vi "AR Drone - Simple Video + Simple nav.vi"() -> ()   [LabVIEW 2014]
doc: "Very simple example showing how to use the base VIs to control the AR Drone and receive and display video data."
uses:
  AR Drone - Simple Video + Simple nav Folder/Control cluster.ctl
  <vilib>/LVH/AR Drone Toolkit/Decode NavData/Typedefs/NavData Demo.ctl
  Global.vi
  <vilib>/LVH/AR Drone Toolkit/AR Drone.lvlib
panel:
  in  "Tab Control 2":enum32{"Setup", "Debug&Test Info", "NavData"}(tab)
  in  "Setup Parameters":T1={"Drone IP address"="192.168.1.1", "Home IP address"="192.168.1.2", "Flight Mode"=enum."INDOOR MODE", "Mounted Hull"=enum."INDOOR HULL", "Video Camera"=1, "Max Altitude (m)"=3.0, "Max Pitch and Roll Angle (deg)"=8.0, "Max Vertical Speed (m/s)"=0.7, "Max Yaw Speed (deg/s)"=100.0} {"Video Camera" items=["Bottom Camera"=1, "Front Camera"=0, "Front in Bottom"=3, "Bottom in Front"=2]}
  in  "device ID":i32=3
  in  "Video Acquisition VI path":path=path "Video Processing.vi"
  in  "Adjustments":cluster{"Sensitivity":dbl, "Null Zone":dbl}={"Sensitivity"=1.0, "Null Zone"=1.0} {"Null Zone" scale=0.0..5.0; "Sensitivity" scale=0.0..5.0}
  out "ctr+nav 2":i32=2242
  in  "milliseconds to wait":u32=10
  out "Refesh Rate (ms)":u32=5
  out "Refesh Rate Video Loop (ms) 2":u32
  in  "video refresh (ms)":u32=40
  out "ctr+nav":errorcluster
  out "NavData Out 2":T2={"control state"=enum."TRANS_LANDING", "battery percentage"=55, "pitch (deg)"=-0.02, "roll (deg)"=0.087, "yaw (deg)"=91.646, "altitude (cm)"=0, "vx (cm/s)?"=0.0, "vy (cm/s)?"=0.0, "vz (cm/s)?"=0.0, "detection cam type"=3}
  out "Battery Remaining 2":dbl(slide)=55.0 scale=0.0..100.0
  out "Hover":bool
  out "Control Cluster":T3={"Roll"=0.0, "Pitch"=-0.10223389, "Vertical Speed"=0.0, "Yaw Speed"=0.0} {"Yaw Speed" scale=-1.0..1.0; "Vertical Speed" scale=-1.0..1.0; "Pitch" scale=-1.0..1.0; "Roll" scale=-1.0..1.0}
  out "error":bool
  out "Take off/Land":bool
  in  "Tab Control":enum32{"Raw Image", "Grayscale", "Black&White"}(tab)
  out "Raw":picture
  out "Grayscale":T4(plugin-control)
  out "B&W":T4(plugin-control)
  in  "Manual":bool=TRUE
  in  "stop":bool
  in  "Emergency Landing":bool
  # "(1 is default)"
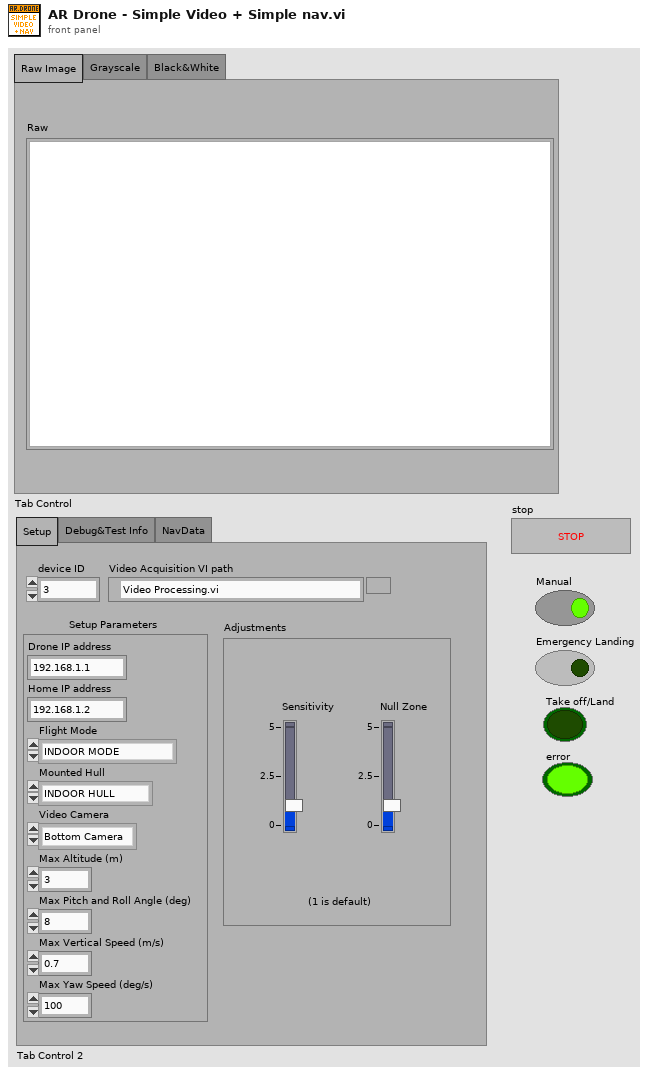
[diagram p1: front panel]
types:
  T1 = cluster{"Drone IP address":string, "Home IP address":string, "Flight Mode":enum8{"OUTDOOR MODE", "INDOOR MODE"}, "Mounted Hull":enum8{"OUTDOOR HULL", "INDOOR HULL"}, "Video Camera":u8, "Max Altitude (m)":sgl, "Max Pitch and Roll Angle (deg)":sgl, "Max Vertical Speed (m/s)":sgl, "Max Yaw Speed (deg/s)":sgl}
  T2 = typedef "AR Drone.lvlib/NavData Demo.ctl" = cluster{"control state":enum32{"DEFAULT", "INIT", "LANDING", "FLYING", "HOVERING", "TEST", "TRANS_TAKEOFF", "TRANS_GOTOFIX", "TRANS_LANDING"}, "battery percentage":u32, "pitch (deg)":sgl, "roll (deg)":sgl, "yaw (deg)":sgl, "altitude (cm)":u32, "vx (cm/s)?":sgl, "vy (cm/s)?":sgl, "vz (cm/s)?":sgl, "detection cam type":u32}
  T3 = typedef "Control cluster.ctl" = cluster{"Roll":sgl, "Pitch":sgl, "Vertical Speed":sgl, "Yaw Speed":sgl}
  T4 = typedef "IMAQ Image.ctl" = refnum<image>
  T5 = typedef "AR Drone.lvlib/AR Drone Resource.ctl" = cluster{"UDP Control Connection":refnum<k16>, "UDP NavData Connection":refnum<k16>, "UDP Video Connection (Drone 1.0)":refnum<k16>, "TCP Video Connection (Drone 2.0)":refnum<k5>, "TCP Control Port Connection":refnum<k5>, "Drone IP address":string, "Drone Command Port":u16, "Drone NavData Port":u16, "Drone Vid Stream Port":u16, "Drone TCP Control Port":u16, "Home IP address":string, "Home Command Port":u16, "Home NavData Port":u16, "Home Vid Stream Port":u16, "Drone Version":i32, "Drone Index":i32, "Command Sequence":i32}
  T6 = cluster{"Hover":bool, "Land/Take off":bool, "button 3":bool, "button 4":bool}
  T7 = cluster{"Roll":dbl, "Pitch":dbl, "Vertical Speed":dbl, "Yaw Speed":dbl}
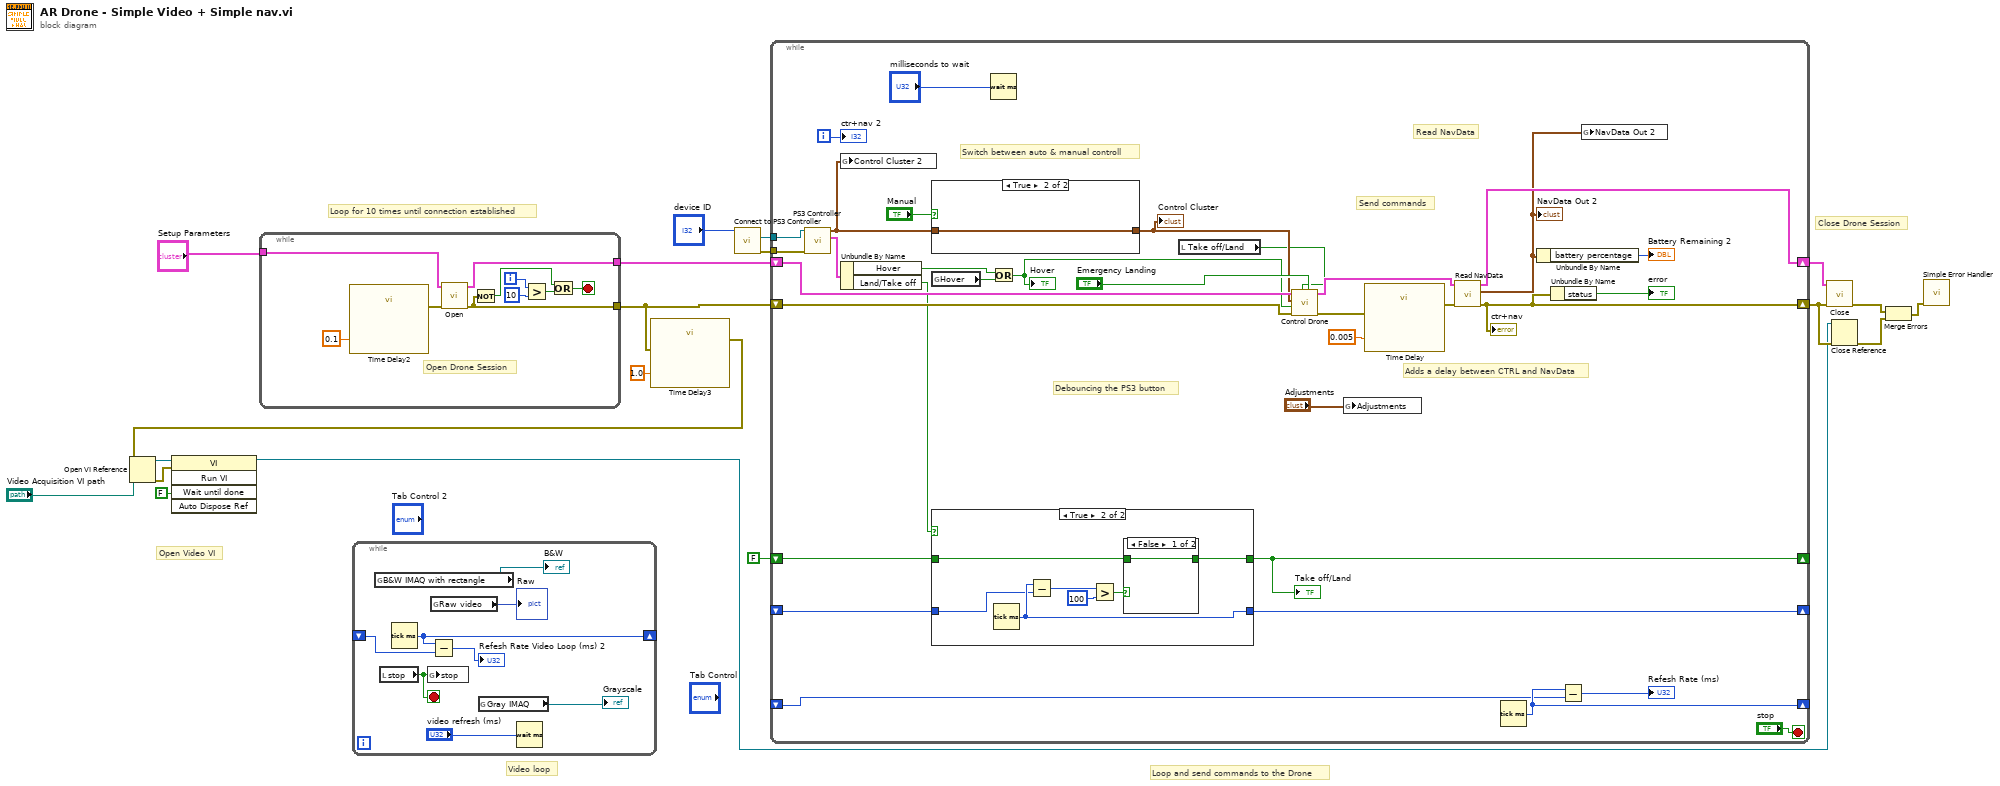
[diagram p0: block diagram]
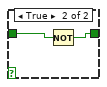
[diagram p3: hidden frame]
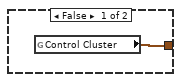
[diagram p4: hidden frame]
diagram:
  # "Open Video VI"
  # "Loop for 10 times until connection established"
  # "Video loop"
  # "Close Drone Session"
  # "Loop and send commands to the Drone"
  n1 = while {
    tunnel: [w21] -> w13
    tunnel: "Setup Parameters" -> [w29]
    tunnel: [w20] -> w5
    i -> [w25]
    stop <- w27 stop-if-true
    # "Open Drone Session"
    n2 = call "Time Delay2"("Delay Time (s)"=0.1) -> ("error out"=w22:errorcluster)  [unwired: 10 in]
    n3 = call <vilib>:"Open.vi"("error in (no error)"=w22, "Setup Parameters"=w29) -> ("error out"=w21:errorcluster, "AR Drone Resource"=w20:T5)  [unwired: 8 in]
    n4 = Not(x=w21) -> (.not. x?=w23:bool)
    n5 = Greater?(x=w25, y=10) -> (0:w26:bool)
    n6 = Or(x=w23, y=w26) -> (x .or. y?=w27:bool)
  }
  n7 = while {
    shift-right: [w35] -> _
    shift-left: _ -> [w34]
    stop <- w31 stop-if-true
    n8 = global read "Global.vi" "B&W IMAQ with rectangle"() -> (→"B&W":T4)
    n9 = local read "stop"() -> (w31:bool)
    n10 = Tick Count (ms)() -> (millisecond timer value=w35:u32)
    n11 = global write "Global.vi" "stop"(w31) -> ()
    n12 = global read "Global.vi" "Raw video"() -> (→"Raw":picture)
    n13 = Subtract(x=w35, y=w34) -> (x-y=→"Refesh Rate Video Loop (ms) 2":u32)
    n14 = global read "Global.vi" "Gray IMAQ"() -> (→"Grayscale":T4)
    n15 = Wait (ms)(milliseconds to wait="video refresh (ms)") -> ()  [unwired: 1 out]
  }
  n16 = call "Time Delay3"("error in (no error)"=w13, "Delay Time (s)"=1.0) -> ("error out"=w1:errorcluster)  [unwired: 9 in]
  n17 = Open VI Reference(vi path="Video Acquisition VI path", error in (no error)=w1) -> (vi reference=w9:refnum<vi>, error out=w7:errorcluster)  [unwired: 4 in]
  n18 = invoke class="VI" method="Run VI"(reference=w9, error in=w7, "Wait until done"=FALSE) -> (reference out=w10:refnum<vi>)  [unwired: 2 in, 4 out]
  n19 = call "Connect to PS3 Controller.vi"("device ID"="device ID") -> ("error out"=w16:errorcluster, "device ID 2"=w18:refnum<k1>)  [unwired: 7 in, 1 out]
  n20 = while {
    shift-right: [w40] -> w19
    shift-left: w5 -> [w68]
    shift-right: [w64] -> w11
    shift-left: w13 -> [w69]
    tunnel: w18 -> [w66]
    tunnel: w16 -> [w65]
    shift-right: [w56] -> _
    shift-left: _ -> [w55]
    shift-right: [w52] -> _
    shift-left: FALSE -> [w53]
    shift-right: [w51] -> _
    shift-left: _ -> [w50]
    i -> [w67]
    stop <- "stop" stop-if-true
    # "Read NavData"
    # "Send commands"
    # "Switch between auto & manual controll"
    # "Debouncing the PS3 button"
    # "Adds a delay between CTRL and NavData"
    n21 = call "PS3 Controller.vi"("error in (no error)"=w65, "device ID"=w66) -> ("Buttons control"=w63:T6, "Control cluster"=w48:T7)  [unwired: 6 in, 2 out]
    n22 = global write "Global.vi" "Control Cluster 2"(w48) -> ()
    n23 = Unbundle By Name(w63) -> ("Hover"=w59:bool, "Land/Take off"=w54:bool)
    n24 = case shown="True" "Manual" {
      tunnel: w48 -> [_ w85]
      tunnel: [w84 w85] -> w49
      frame False {
        n25 = global read "Global.vi" "Control Cluster"() -> (w84:T3)
      }
      frame True {
      }
    }
    "Control Cluster" <- w49
    n26 = global read "Global.vi" "Hover"() -> (w58:bool)
    n27 = case shown="True" w54 {
      tunnel: [w73 w74] -> w52
      tunnel: w53 -> [w73 w75]
      tunnel: [w72 w80] -> w51
      tunnel: w50 -> [w72 w79]
      frame False {
      }
      frame True {
        n28 = Tick Count (ms)() -> (millisecond timer value=w80:u32)
        n29 = Subtract(x=w80, y=w79) -> (x-y=w78:u32)
        n30 = Greater?(x=w78, y=u32 100) -> (0:w76:bool)
        n31 = case shown="False" w76 {
          tunnel: w75 -> [w81 w83]
          tunnel: [w81 w82] -> w74
          frame False {
          }
          frame True {
            n32 = Not(x=w83) -> (.not. x?=w82:bool)
          }
        }
      }
    }
    "Take off/Land" <- w52
    n33 = Wait (ms)(milliseconds to wait="milliseconds to wait") -> ()  [unwired: 1 out]
    n34 = Or(x=w59, y=w58) -> (x .or. y?=w57:bool)
    "Hover" <- w57
    n35 = local read "Take off/Land"() -> (w41:bool)
    n36 = call <vilib>:"Control Drone.vi"("Emergency Landing"="Emergency Landing", "Takeoff/Land"=w41, "error in (no error)"=w69, "Hover"=w57, "Control Cluster"=w49, "AR Drone Resource"=w68) -> ("error out"=w45:errorcluster, "AR Drone Resource Out"=w62:T5)  [unwired: 4 in]
    n37 = global write "Global.vi" "Adjustments"("Adjustments") -> ()
    n38 = call "Time Delay"("error in (no error)"=w45, "Delay Time (s)"=0.005) -> ("error out"=w44:errorcluster)  [unwired: 9 in]
    n39 = call <vilib>:"Read NavData.vi"("error in (no error)"=w44, "AR Drone Resource"=w62) -> ("error out"=w64:errorcluster, "NavData Out"=w39:T2, "AR Drone Resource Out"=w40:T5)  [unwired: 7 in]
    "ctr+nav" <- w64
    "NavData Out 2" <- w39
    n40 = Tick Count (ms)() -> (millisecond timer value=w56:u32)
    n41 = Unbundle By Name(w39) -> ("battery percentage"=→"Battery Remaining 2":u32)
    n42 = Unbundle By Name(w64) -> ("status"=→"error":bool)
    n43 = Subtract(x=w56, y=w55) -> (x-y=→"Refesh Rate (ms)":u32)
    n44 = global write "Global.vi" "NavData Out 2"(w39) -> ()
    "ctr+nav 2" <- w67
  }
  n45 = call <vilib>:"Close.vi"("error in (no error)"=w11, "AR Drone Resource"=w19) -> ("error out"=w4:errorcluster)  [unwired: 9 in]
  n46 = Close Reference(reference=w10, error in (no error)=w11) -> (error out=w3:errorcluster)
  n47 = Merge Errors(w4, w3) -> (w2:errorcluster)
  n48 = call <vilib>:"Simple Error Handler.vi"("error in (no error)"=w2) -> ()  [unwired: 4 in, 5 out]
